vi "Alerte Debit compteurs.vi"() -> ()   [LabVIEW 2022 SP3]
uses:
  Enum/Enum 2.ctl
  Variables globales/Variable globale compteurs.vi
  Variables globales/Variable glob alertes Compteurs.vi
panel:
  out "Nb pages":u8
  in  "ajouter":bool
  in  "Groupes":T1(array[cluster])=[{"valeur alerte"=1000.0, "Alerte"=FALSE, "Indices a controler"=[5], "N°"=0}] caption="Groupes alertes debits compteurs" {"valeur alerte" min=1e-07 max=1000.0 step=1e-07}
  in  "OK":bool
  in  "Annuler":bool
  # "PARAMETRES POUR ALERTE sur \ndebit compteur PAR ENVOI D'UN MAIL"
  # "Ce logiciel et les informations qu'il contient, sont la propriété de l’IAS et ne peuvent être diffusés sans l’autorisation de la Station d’étalonnage"
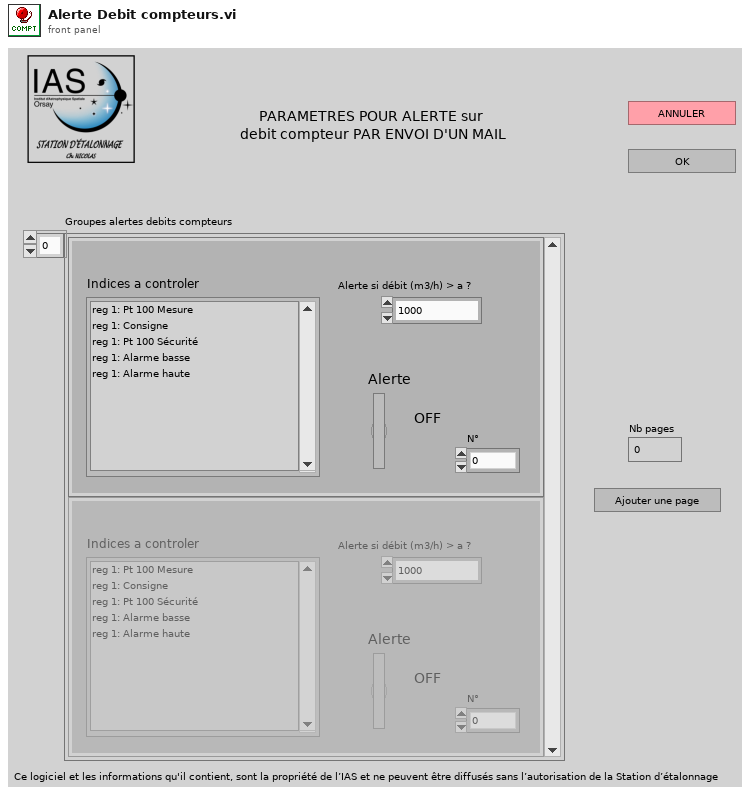
[diagram p1: front panel]
types:
  T1 = cluster{"valeur alerte":dbl, "Alerte":bool, "Indices a controler":i32[], "N°":u16}[]
  T2 = typedef "Enum 2.ctl" = enum16{"init noms", "initialisation", "choix", "GO"}
  T3 = cluster{"Nom tache compteurs":refnum<k21>, "Noms des compteurs":string[], "Selection":bool[], "Init compteurs":dbl[], "Noms compteurs selectionnes":string[]}
  T4 = cluster{"Alerte":bool, "valeur alerte":dbl, "Défaut":bool, "Indices à controler":i16[], "N°":u16}[]
  T5 = cluster{"valeur alerte":dbl, "Alerte":bool, "Indices a controler":i32[], "N°":u16}
  T6 = cluster{"Alerte":bool, "valeur alerte":dbl, "Défaut":bool, "Indices à controler":i16[], "N°":u16}
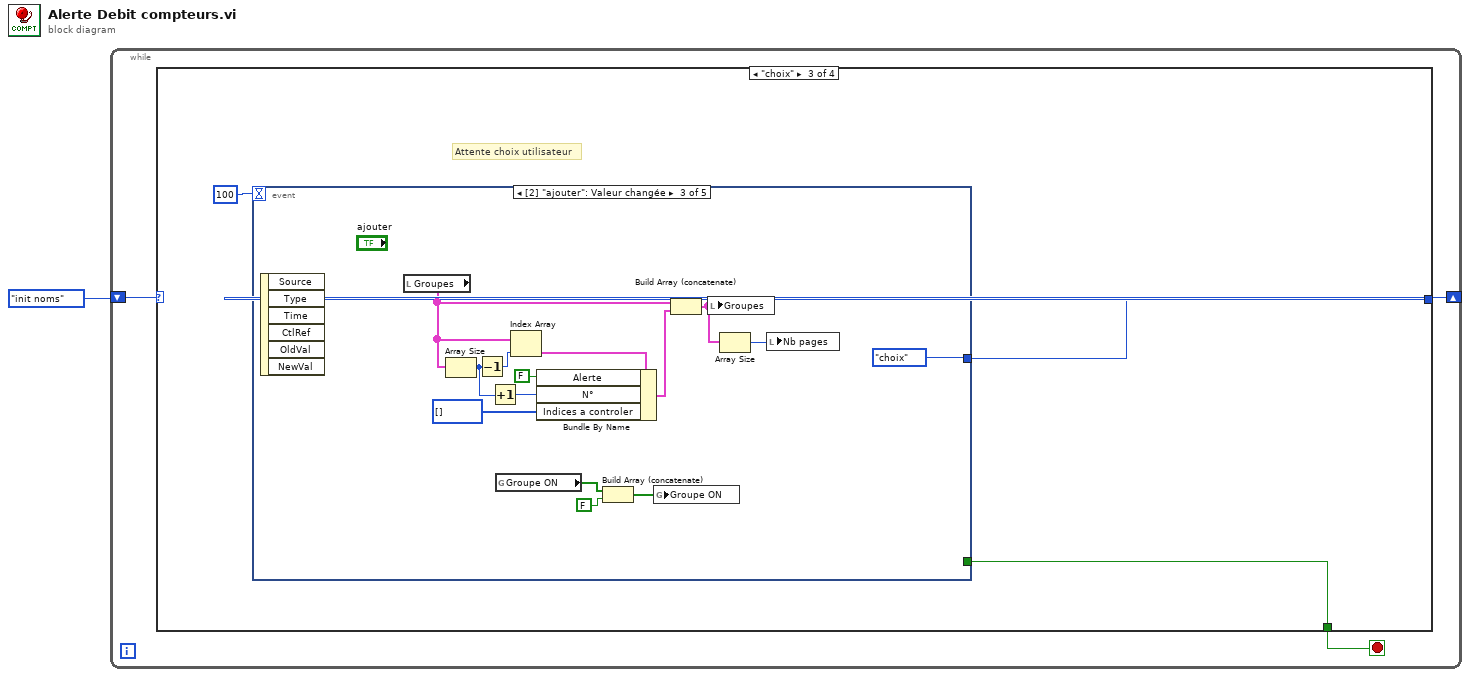
[diagram p0: block diagram]
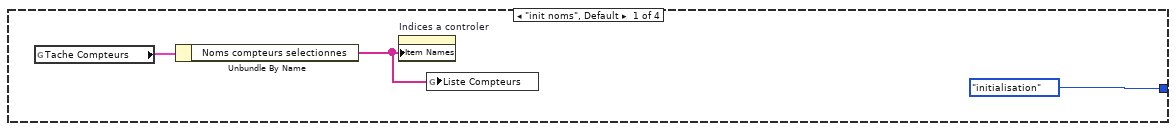
[diagram p2: hidden frame]
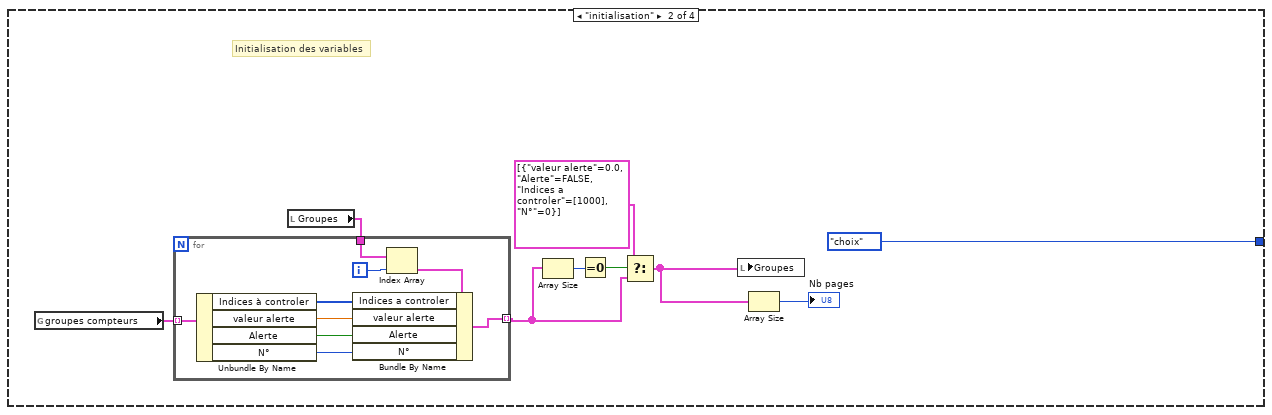
[diagram p3: hidden frame]
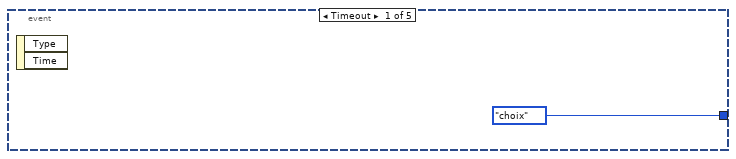
[diagram p4: hidden frame]
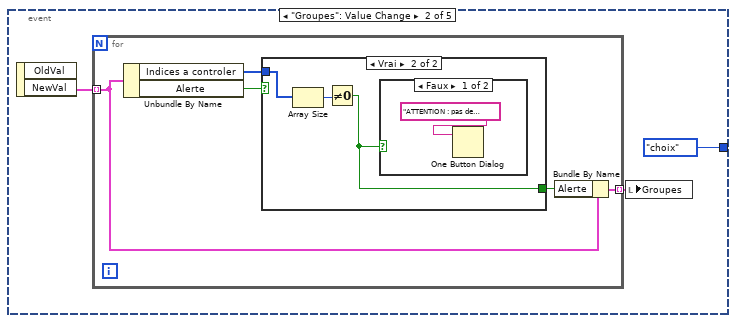
[diagram p5: hidden frame]
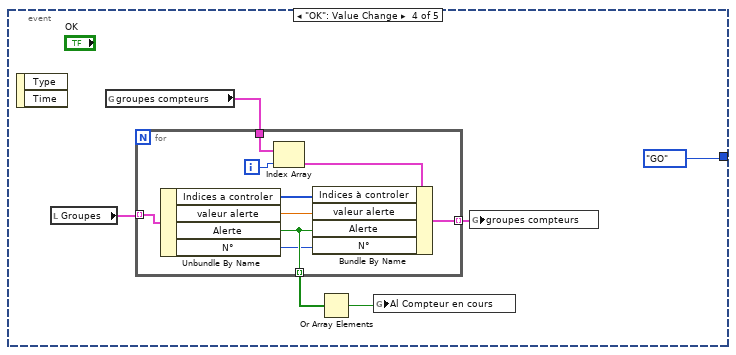
[diagram p8: hidden frame]
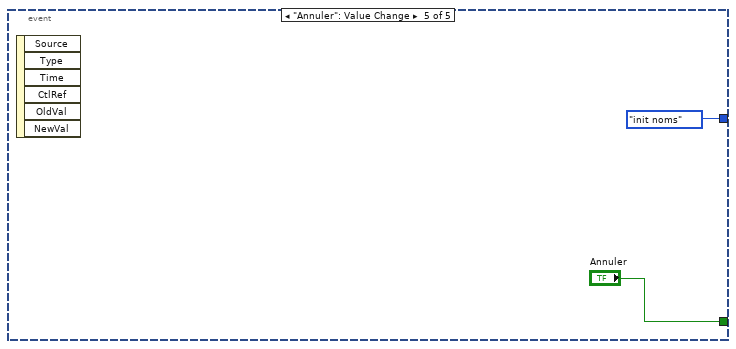
[diagram p9: hidden frame]
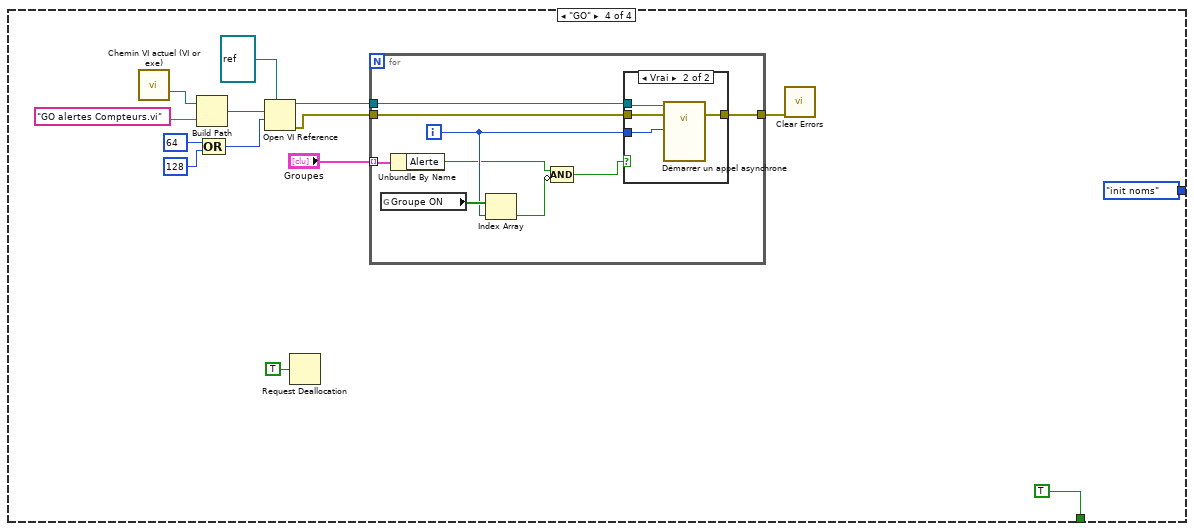
[diagram p10: hidden frame]
diagram:
  n1 = while {
    shift-right: [w3] -> _
    shift-left: Enum_2."init noms" ("Énum") -> [w4]
    stop <- w2 stop-if-true
    n2 = case shown="\"choix\"" w4 {
      tunnel: [Enum_2."initialisation" ("Énum") Enum_2."choix" ("Énum") w26 Enum_2."init noms" ("Énum")] -> w3
      tunnel: [_ _ w27 TRUE] -> w2
      frame "init noms", Default {
        n3 = global read "Variable globale compteurs.vi" "Tache Compteurs"() -> (w7:T3)
        n4 = Unbundle By Name(w7) -> ("Noms compteurs selectionnes"=w5:string[])
        n5 = property on="Indices a controler" class="LstDér (strict)"("Item Names"=w5) -> ()  [unwired: 2 in, 2 out]
        n6 = global write "Variable glob alertes Compteurs.vi" "Liste Compteurs"(w5) -> ()
      }
      frame "initialisation" {
        # "Initialisation des variables"
        n7 = global read "Variable glob alertes Compteurs.vi" "groupes compteurs"() -> (w15:T4)
        n8 = local read "Groupes"() -> (w14:T1)
        n9 = for {
          tunnel: w15 -> [w25] mode=indexing
          tunnel: w14 -> [w24]
          tunnel: [w18] -> w11 mode=indexing
          i -> [w23]
          n10 = Unbundle By Name(w25) -> ("Indices à controler"=w21:i16[], "valeur alerte"=w20:dbl, "Alerte"=w19:bool, "N°"=w17:u16)
          n11 = Index Array(array=w24, index=w23) -> (element=w22:T5)
          n12 = Bundle By Name(cluster=w22, "Indices a controler"=w21, "valeur alerte"=w20, "Alerte"=w19, "N°"=w17) -> (w18:T5)
        }
        n13 = Array Size(array=w11) -> (size(s)=w12:i32)
        n14 = Equal To 0?(x=w12) -> (x = 0?=w13:bool)
        n15 = Select(t=T1 [{"valeur alerte"=0.0, "Alerte"=FALSE, "Indices a controler"=[1000], "N°"=0}] ("cas vrai"), s=w13, f=w11) -> (s? t:f=w10:T1)
        n16 = local write "Groupes"(w10) -> ()
        n17 = Array Size(array=w10) -> (size(s)=→"Nb pages":i32)
      }
      frame "choix" {
        # "Attente choix utilisateur"
        n18 = event shown="[2] \"ajouter\": Valeur changée" {
          selector: _ -> [_ _ _ _ _]
          dyn-events: _ -> [_ _ _ _ _]
          timeout: 100 -> [_ _ _ _ _]
          tunnel: [_ _ _ _ "Annuler"] -> w27
          tunnel: [Enum_2."choix" ("Énum") Enum_2."choix" ("Énum") Enum_2."choix" ("Énum") Enum_2."GO" ("Énum") Enum_2."init noms" ("Énum")] -> w26
          event Timeout {
            n19 = event-data() -> ()  [unwired: 1 in, 2 out]
          }
          event "Groupes": Value Change {
            n20 = event-data() -> ("NewVal"=w32:T1)  [unwired: 1 in, 1 out]
            n21 = for {
              tunnel: w32 -> [w36] mode=indexing
              tunnel: [w33] -> w31 mode=indexing
              n22 = Unbundle By Name(w36) -> ("Indices a controler"=w35:i32[], "Alerte"=w37:bool)
              n23 = case shown="Vrai" w37 {
                selector: w37 -> [w38 _]
                tunnel: w35 -> [_ w41]
                tunnel: [w38 w39] -> w34
                frame False {
                }
                frame True {
                  n24 = Array Size(array=w41) -> (size(s)=w40:i32)
                  n25 = Not Equal To 0?(x=w40) -> (x != 0?=w39:bool)
                  n26 = case shown="Faux" w39 {
                    frame False {
                      n27 = One Button Dialog(message="ATTENTION : pas de capteur choisi dans la liste") -> ()  [unwired: 1 in, 1 out]
                    }
                    frame True {
                    }
                  }
                }
              }
              n28 = Bundle By Name(cluster=w36, "Alerte"=w34) -> (w33:T5)
            }
            n29 = local write "Groupes"(w31) -> ()
          }
          event "ajouter": Value Change {
            n30 = event-data() -> ()  [unwired: 1 in, 6 out]
            n31 = local read "Groupes"() -> (w53:T1)
            n32 = Array Size(array=w53) -> (size(s)=w45:i32)
            n33 = Decrement(x=w45) -> (x-1=w52:i32)
            n34 = Increment(x=w45) -> (x+1=w44:i32)
            n35 = global read "Variable glob alertes Compteurs.vi" "Groupe ON"() -> (w48:bool[])
            n36 = Index Array(array=w53, index=w52) -> (element=w54:T5)
            n37 = Bundle By Name(cluster=w54, "Alerte"=FALSE, "N°"=w44, "Indices a controler"=i32[] []) -> (w56:T5)
            n38 = Build Array (concatenate)(w48, FALSE) -> (w47:bool[])
            n39 = global write "Variable glob alertes Compteurs.vi" "Groupe ON"(w47) -> ()
            n40 = Build Array (concatenate)(w53, w56) -> (w50:T1)
            n41 = local write "Groupes"(w50) -> ()
            n42 = Array Size(array=w50) -> (size(s)=w49:i32)
            n43 = local write "Nb pages"(w49) -> ()
          }
          event "OK": Value Change {
            n44 = event-data() -> ()  [unwired: 1 in, 2 out]
            n45 = local read "Groupes"() -> (w61:T1)
            n46 = global read "Variable glob alertes Compteurs.vi" "groupes compteurs"() -> (w62:T4)
            n47 = for {
              tunnel: w61 -> [w71] mode=indexing
              tunnel: w62 -> [w70]
              tunnel: [w65] -> w60 mode=indexing
              tunnel: [w64] -> w59 mode=indexing
              i -> [w69]
              n48 = Unbundle By Name(w71) -> ("Indices a controler"=w67:i32[], "valeur alerte"=w66:dbl, "Alerte"=w64:bool, "N°"=w63:u16)
              n49 = Index Array(array=w70, index=w69) -> (element=w68:T6)
              n50 = Bundle By Name(cluster=w68, "Indices à controler"=w67, "valeur alerte"=w66, "Alerte"=w64, "N°"=w63) -> (w65:T6)
            }
            n51 = Or Array Elements(Boolean array=w59) -> (logical OR=w58:bool)
            n52 = global write "Variable glob alertes Compteurs.vi" "Al Compteur en cours"(w58) -> ()
            n53 = global write "Variable glob alertes Compteurs.vi" "groupes compteurs"(w60) -> ()
          }
          event "Annuler": Value Change {
            n54 = event-data() -> ()  [unwired: 1 in, 6 out]
          }
        }
      }
      frame "GO" {
        n55 = call "Chemin VI actuel (VI or exe).vi"() -> ("VI or executable installation directory"=w80:path)  [unwired: 14 in, 1 out]
        n56 = Build Path(base path=w80, name or relative path="GO alertes Compteurs.vi" ("nom ou chemin relatif")) -> (appended path=w76:path)
        n57 = Compound Arithmetic op=OR(64 ("options"), 128 ("options")) -> (w79:i32)
        n58 = Open VI Reference(type specifier VI Refnum (for type only)=refnum<vi> refnum ("spécificateur de type du refnum de VI (pour type seulement)"), vi path=w76, options=w79) -> (vi reference=w81:refnum<vi>, error out=w82:errorcluster)  [unwired: 3 in]
        n59 = Request Deallocation(TRUE ("flag")) -> ()
        n60 = for {
          tunnel: w81 -> [w94]
          tunnel: w82 -> [w96]
          tunnel: [w95] -> w84
          tunnel: "Groupes" -> [w93] mode=indexing
          i -> [w91]
          n61 = global read "Variable glob alertes Compteurs.vi" "Groupe ON"() -> (w92:bool[])
          n62 = Unbundle By Name(w93) -> ("Alerte"=w90:bool)
          n63 = Index Array(array=w92, index=w91) -> (element=w89:bool)
          n64 = Compound Arithmetic op=AND ("Opérateur arithmétique")(w90, invert w89) -> (w88:bool)
          n65 = case shown="Vrai" w88 {
            tunnel: w96 -> [w97 w101]
            tunnel: [w97 w100] -> w95
            tunnel: w94 -> [_ w98]
            tunnel: w91 -> [_ w99]
            frame False {
            }
            frame True {
              n66 = call-by-ref "Démarrer un appel asynchrone"(reference=w98, error in=w101, "Numéro"=w99) -> (error out=w100:errorcluster)  [unwired: 5 in, 1 out]
            }
          }
        }
        n67 = call <vilib>:"Clear Errors.vi"("error in (no error)"=w84) -> ()  [unwired: 5 in, 2 out]
      }
    }
  }
